vi "Cmd HO.vi"(8 "error in (no error)":errorcluster caption="에러 입력(에러 없음)", 11 "CO3000 입력":refnum<class "CO3000.lvclass">) -> (0 "error out":errorcluster caption="에러 출력", 3 "CO3000 출력":refnum<class "CO3000.lvclass">)   [LabVIEW 2023, in "Turn Table and Mast.lvlib" / "CO3000.lvclass"]
uses:
  CO3000.lvclass
  CO3000.lvclass/CO3000.ctl
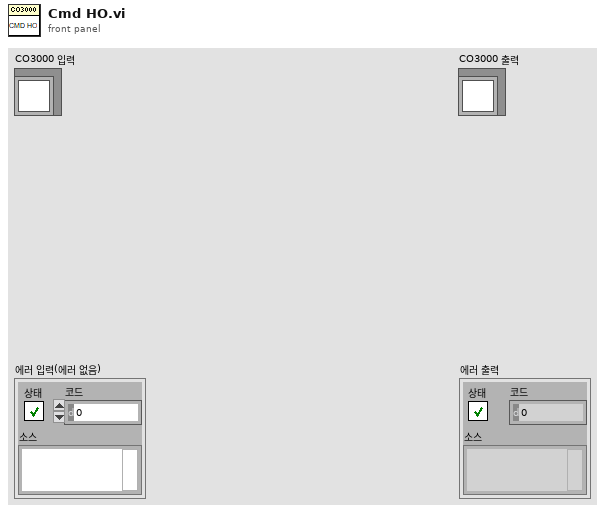
[diagram p1: front panel]
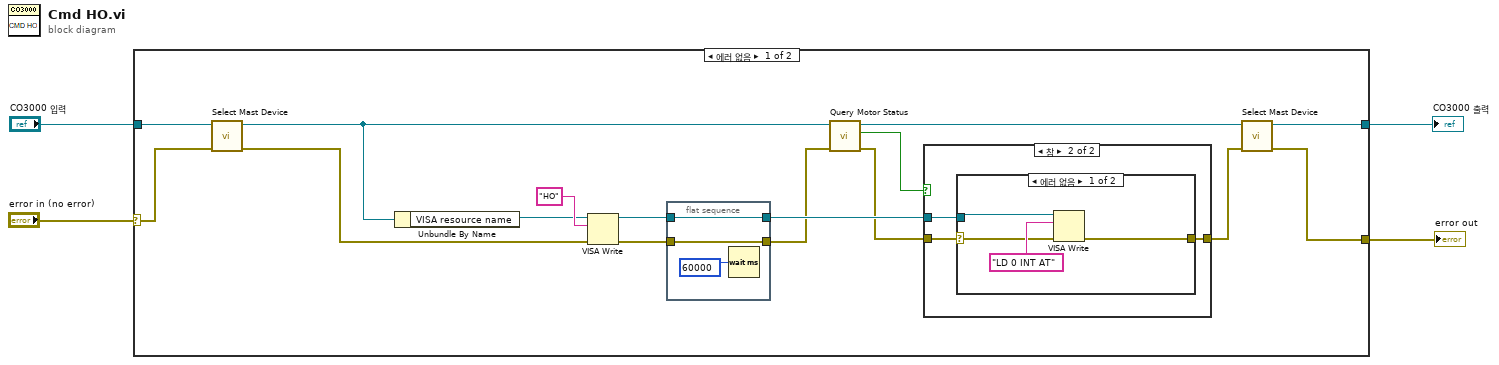
[diagram p0: block diagram]
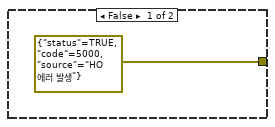
[diagram p2: hidden frame]
diagram:
  n1 = case shown="에러 없음" "error in (no error)" {
    selector: "error in (no error)" -> [w15 w34]
    tunnel: "CO3000 입력" -> [w16 w33]
    tunnel: [w5 w34] -> w1
    tunnel: [w7 w33] -> w3
    frame No Error {
      n2 = call "Select Mast Device.vi"("error in (no error)"=w15, "CO3000 in"=w16) -> ("error out"=w12:errorcluster, "CO3000 out"=w14:refnum<class "CO3000.lvclass">)  [unwired: 8 in]
      n3 = Unbundle By Name(w14) -> ("VISA resource name"=w13:refnum<visa-resource-name>)
      n4 = VISA Write(VISA resource name=w13, write buffer="HO" ("버퍼 쓰기"), error in (no error)=w12) -> (VISA resource name out=w19:refnum<visa-resource-name>, error out=w18:errorcluster)  [unwired: 1 out]
      n5 = flat-sequence {
        tunnel: w18 -> [w31]
        tunnel: w19 -> [w30]
        tunnel: [w31] -> w11
        tunnel: [w30] -> w17
        frame #0 {
          n6 = Wait (ms)(milliseconds to wait=u32 60000 ("대기 시간 (ms)")) -> ()  [unwired: 1 out]
        }
      }
      n7 = call-dynamic "Query Motor Status.vi"("error in (no error)"=w11, "CO3000 in"=w14) -> ("error out"=w10:errorcluster, "Motor Stop?"=w9:bool, "CO3000 out"=w8:refnum<class "CO3000.lvclass">)  [unwired: 7 in]
      n8 = case shown="참" w9 {
        tunnel: w17 -> [_ w24]
        tunnel: [errorcluster {"status"=TRUE, "code"=5000, "source"="HO 에러 발생"} ("에러 상수") w23] -> w6
        tunnel: w10 -> [_ w22]
        frame False {
        }
        frame True {
          n9 = case shown="에러 없음" w22 {
            selector: w22 -> [w26 w29]
            tunnel: w24 -> [w27 _]
            tunnel: [w25 w29] -> w23
            frame No Error {
              n10 = VISA Write(VISA resource name=w27, write buffer="LD 0 INT AT" ("버퍼 쓰기"), error in (no error)=w26) -> (error out=w25:errorcluster)  [unwired: 2 out]
            }
            frame Error {
            }
          }
        }
      }
      n11 = call "Select Mast Device.vi"("error in (no error)"=w6, "CO3000 in"=w8) -> ("error out"=w5:errorcluster, "CO3000 out"=w7:refnum<class "CO3000.lvclass">)  [unwired: 8 in]
    }
    frame Error {
    }
  }
  "error out" <- w1
  "CO3000 출력" <- w3
